vi "SeqEditor_init-Frist.vi"(8 "error in (no error)":errorcluster, 11 "NLTest in":refnum<class "NLTest.lvclass">) -> (0 "error out":errorcluster, 3 "NLTest out":refnum<class "NLTest.lvclass">)   [LabVIEW 2017, in "NLTest.lvclass"]
uses:
  NLTest.lvclass
  <vilib>/Utility/miscctls.llb/LVPointTypeDef.ctl
  <vilib>/Utility/miscctls.llb/LVRowAndColumnTypeDef.ctl
  NLTest.lvclass/NLTest.ctl
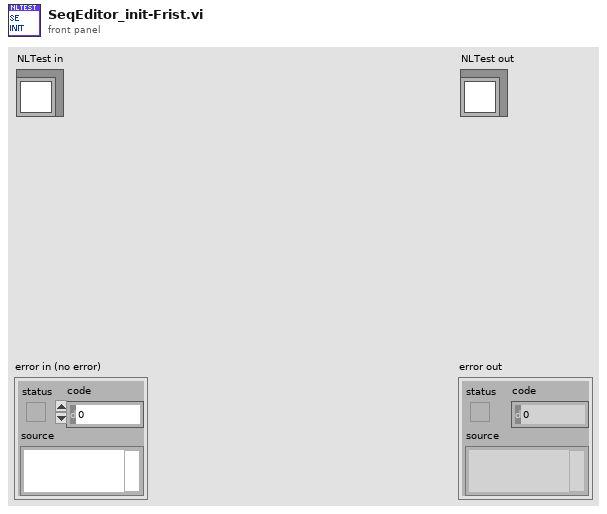
[diagram p1: front panel]
types:
  T1 = typedef "LVRowAndColumnTypeDef.ctl" = cluster{"Row":i32, "Column":i32}
  T2 = typedef "LVPointTypeDef.ctl" = cluster{"Horizontal":i16, "Vertical":i16}
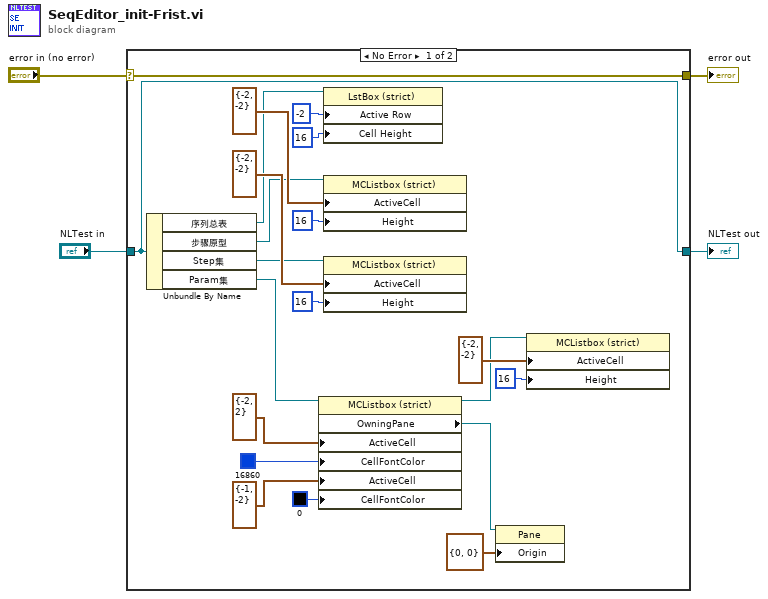
[diagram p0: block diagram]
diagram:
  n1 = case shown="No Error" "error in (no error)" {
    selector: "error in (no error)" -> [w25 w27]
    tunnel: [w25 w27] -> w3
    tunnel: [w24 w26] -> w1
    tunnel: "NLTest in" -> [w24 w26]
    frame No Error {
      n2 = Unbundle By Name(w24) -> ("序列总表"=w8:refnum<vi>, "步骤原型"=w7:refnum<vi>, "Step集"=w6:refnum<vi>, "Param集"=w23:refnum<vi>)
      n3 = property class="MCListbox (strict)"(reference=w23, "ActiveCell"=T1 {"Row"=-2, "Column"=2} ("Active Cell:Active Cell"), "CellFontColor"=u32 16860, "ActiveCell"=T1 {"Row"=-1, "Column"=-2} ("Active Cell:Active Cell"), "CellFontColor"=u32 0) -> (reference out=w5:refnum<vi>, "OwningPane"=w22:refnum<vi>)  [unwired: 1 in, 1 out]
      n4 = property on="Property Node" class="LstBox (strict)"(reference=w8, "Active Row"=-2 ("Active Row:Active Row Number"), "Cell Height"=u32 16 ("Active Cell:Cell Size:Height")) -> ()  [unwired: 1 in, 2 out]
      n5 = property on="Property Node" class="MCListbox (strict)"(reference=w7, "ActiveCell"=T1 {"Row"=-2, "Column"=-2} ("Active Cell:Active Cell"), "Height"=u32 16 ("Active Cell:Cell Size:Height")) -> ()  [unwired: 1 in, 2 out]
      n6 = property on="Property Node" class="MCListbox (strict)"(reference=w6, "ActiveCell"=T1 {"Row"=-2, "Column"=-2} ("Active Cell:Active Cell"), "Height"=u32 16 ("Active Cell:Cell Size:Height")) -> ()  [unwired: 1 in, 2 out]
      n7 = property class="Pane"(reference=w22, "Origin"=T2 {"Horizontal"=0, "Vertical"=0}) -> ()  [unwired: 1 in, 2 out]
      n8 = property on="Property Node" class="MCListbox (strict)"(reference=w5, "ActiveCell"=T1 {"Row"=-2, "Column"=-2} ("Active Cell:Active Cell"), "Height"=u32 16 ("Active Cell:Cell Size:Height")) -> ()  [unwired: 1 in, 2 out]
    }
    frame Error {
    }
  }
  "error out" <- w3
  "NLTest out" <- w1
